vi "niDAQmx Initialize gRPC Task.vi"(8 "error in":errorcluster, 10 "gRPC options":T1={"task name"="", "address (localhost)"="localhost", "port (31763)"=31763}, 11 "task name":string) -> (0 "error out":errorcluster, 3 "task out":refnum<class "Session Factory.lvclass">)   [LabVIEW 2021, in "Session Management niDAQmx.lvlib" / "Session Factory.lvclass"]
doc: "Initializes the niDAQmx task on the specified NI gRPC Device Server. Returns a session factory object to be used in all subsequent niDAQmx client wrapper VI calls."
uses:
  Session Factory.lvclass
  niDAQmx gRPC Device Server.ctl
  NI DAQmx Client/RPC Messages/nidaqmx_grpc_CreateTaskRequest.ctl
  NI DAQmx Client/RPC Messages/nidevice_grpc_SessionInitializationBehavior.ctl
  Session Factory.lvclass/Session Factory.ctl
  NI DAQmx Client/NI_DAQmx_client.lvlib
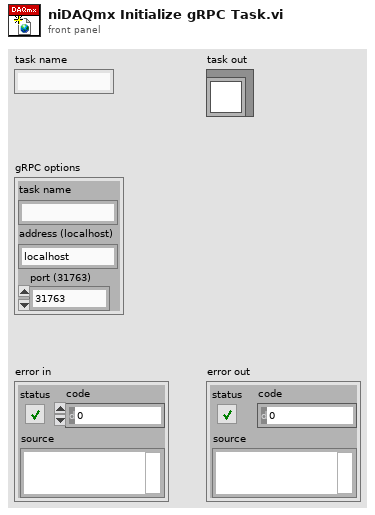
[diagram p1: front panel]
types:
  T1 = typedef "Session Management niDAQmx.lvlib/Session Factory.lvclass/niDAQmx gRPC Device Server.ctl" = cluster{"task name":string, "address (localhost)":string, "port (31763)":u32}
  T2 = typedef "NI_DAQmx_client.lvlib/nidevice_grpc_SessionInitializationBehavior.ctl" = enum32{"SESSION_INITIALIZATION_BEHAVIOR_UNSPECIFIED", "SESSION_INITIALIZATION_BEHAVIOR_INITIALIZE_NEW", "SESSION_INITIALIZATION_BEHAVIOR_ATTACH_TO_EXISTING"}
  T3 = typedef "NI_DAQmx_client.lvlib/nidaqmx_grpc_CreateTaskRequest.ctl" = cluster{"session_name":string, "initialization_behavior":T2}
  T4 = typedef "grpc-lvsupport-release.lvlib/grpcId.ctl" = u64
  T5 = typedef "NI_DAQmx_client.lvlib/nidaqmx_grpc_CreateTaskResponse.ctl" = cluster{"status":i32, "task":T6, "new_session_initialized":bool}
  T6 = typedef "NI_DAQmx_client.lvlib/nidevice_grpc_Session.ctl" = cluster{"nidevice_grpc_Session_session":refnum<class "nidevice_grpc_Session_session.lvclass">}
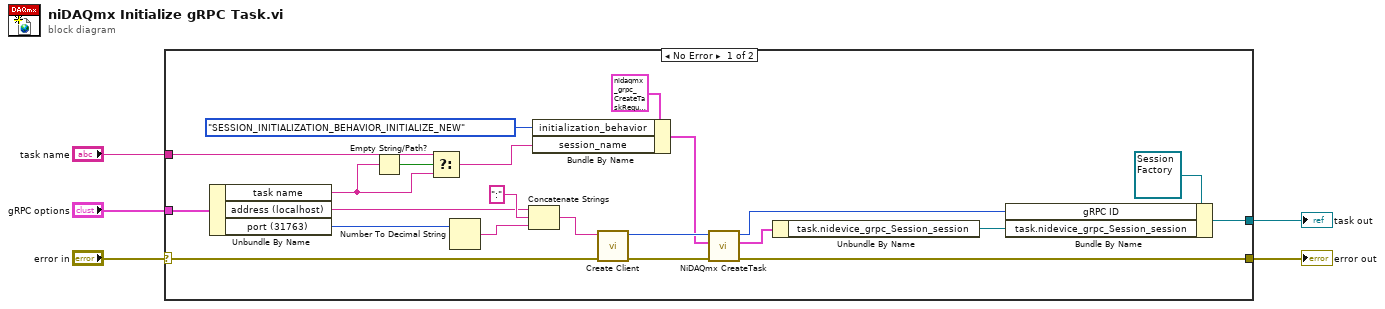
[diagram p0: block diagram]
diagram:
  n1 = case shown="No Error" "error in" {
    selector: "error in" -> [w20 w28]
    tunnel: [w25 w28] -> w4
    tunnel: "task name" -> [w8 _]
    tunnel: [w16 _] -> w2
    tunnel: "gRPC options" -> [w14 _]
    frame No Error {
      n2 = Unbundle By Name(w14) -> ("task name"=w7:string, "address (localhost)"=w12:string, "port (31763)"=w13:u32)
      n3 = Empty String/Path?(string/path=w7) -> (empty?=w9:bool)
      n4 = Select(t=w8, s=w9, f=w7) -> (s? t:f=w6:string)
      n5 = Number To Decimal String(number=w13) -> (decimal integer string=w11:string)  [unwired: 1 in]
      n6 = Concatenate Strings(w12, ":" ("string"), w11) -> (w23:string)
      n7 = Bundle By Name(cluster=T3 {"session_name"="", "initialization_behavior"=enum."SESSION_INITIALIZATION_BEHAVIOR_INITIALIZE_NEW"} ("Request Data"), "initialization_behavior"=nidevice_grpc_SessionInitializationBehavior."SESSION_INITIALIZATION_BEHAVIOR_INITIALIZE_NEW", "session_name"=w6) -> (w21:T3)
      n8 = call "Create Client.vi"("error in"=w20, "address"=w23) -> ("error out"=w27:errorcluster, "gRPC ID Out"=w26:T4)  [unwired: 8 in]
      n9 = call "NiDAQmx CreateTask.vi"("error in"=w27, "Request Data"=w21, "gRPC ID"=w26) -> ("error out"=w25:errorcluster, "Response Data"=w18:T5, "gRPC ID out"=w19:T4)  [unwired: 6 in]
      n10 = Unbundle By Name(w18) -> ("task.nidevice_grpc_Session_session"=w17:refnum<class "nidevice_grpc_Session_session.lvclass">)
      n11 = Bundle By Name(cluster=refnum<class "Session Factory.lvclass"> refnum ("session factory out"), "gRPC ID"=w19, "task.nidevice_grpc_Session_session"=w17) -> (w16:refnum<class "Session Factory.lvclass">)
    }
    frame Error {
    }
  }
  "error out" <- w4
  "task out" <- w2
